vi "Build CE Deploy - Create Project.vi"(8 "error in":errorcluster, 10 "Project Files":path[](array[path]), 11 "Target Dir":path) -> (0 "error out":errorcluster, 2 "Project File Path":path, 3 "dup Target Dir":path)   [LabVIEW 2021]
doc: "::: CalcExpress Toolkit :::\nCopyright (c) 2000-2026 Konstantin Shifershteyn. All rights reserved."
panel:
  # "CalcExpress Toolkit\nCopyright (c) 2000-2026 Konstantin Shifershteyn"
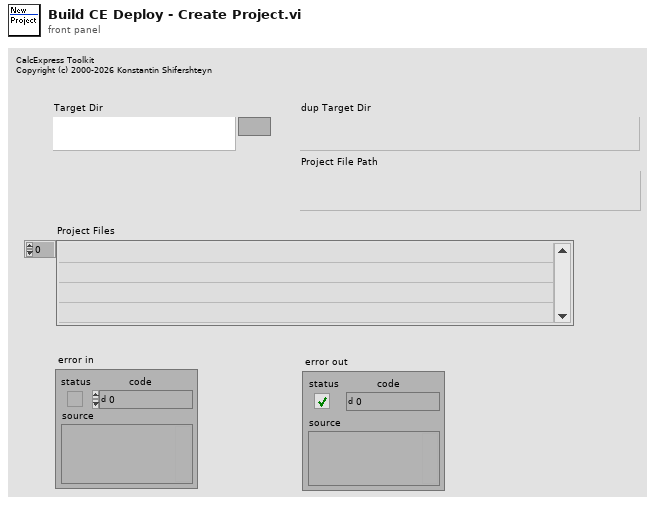
[diagram p1: front panel]
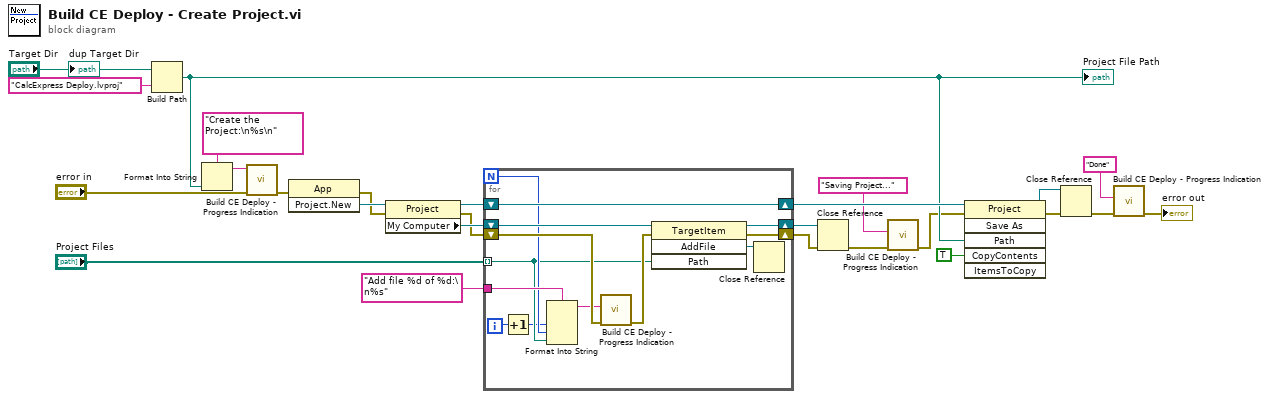
[diagram p0: block diagram]
diagram:
  n1 = Build Path(base path="Target Dir", name or relative path="CalcExpress Deploy.lvproj") -> (appended path=w7:path)
  "Project File Path" <- w7
  n2 = Format Into String(format string="Create the Project:\n%s\n", w7) -> (resulting string=w9:string)  [unwired: 2 in, 1 out]
  n3 = call "Build CE Deploy - Progress Indication.vi"("error in"="error in", "message 1"=w9) -> ("error out"=w11:errorcluster)  [unwired: 9 in]
  n4 = invoke class="App" method="Project.New"(error in=w11) -> (error out=w22:errorcluster, "Project:New"=w24:refnum<vi>)  [unwired: 2 in, 1 out]
  n5 = property class="Project"(reference=w24, error in=w22) -> (reference out=w26:refnum<vi>, error out=w20:errorcluster, "My Computer"=w23:refnum<vi>)
  n6 = for {
    N -> [w30]
    tunnel: "Project Files" -> [w29] mode=indexing
    shift-right: [w38] -> w21
    shift-left: w23 -> [w39]
    shift-right: [w36] -> w25
    shift-left: w20 -> [w34]
    shift-right: [w35] -> w14
    shift-left: w26 -> [w35]
    tunnel: "Add file %d of %d:\n%s" -> [w32]
    i -> [w31]
    n7 = Increment(x=w31) -> (x+1=w28:i32)
    n8 = Format Into String(format string=w32, w28, w30, w29) -> (resulting string=w27:string)  [unwired: 2 in, 1 out]
    n9 = call "Build CE Deploy - Progress Indication.vi"("error in"=w34, "message 2"=w27) -> ("error out"=w33:errorcluster)  [unwired: 9 in]
    n10 = invoke class="TargetItem" method="AddFile"(reference=w39, error in=w33, "Path"=w29) -> (reference out=w38:refnum<vi>, error out=w36:errorcluster, "AddFile"=w37:refnum<vi>)  [unwired: 1 in, 1 out]
    n11 = Close Reference(reference=w37) -> ()  [unwired: 1 in, 1 out]
  }
  n12 = Close Reference(reference=w21, error in (no error)=w25) -> (error out=w6:errorcluster)
  n13 = call "Build CE Deploy - Progress Indication.vi"("error in"=w6, "message 2"="Saving Project...") -> ("error out"=w5:errorcluster)  [unwired: 9 in]
  n14 = invoke class="Project" method="Save As"(reference=w14, error in=w5, "Path"=w7, "CopyContents"=TRUE ("Copy contents?")) -> (reference out=w17:refnum<vi>, error out=w18:errorcluster)  [unwired: 2 in, 4 out]
  n15 = Close Reference(reference=w17, error in (no error)=w18) -> (error out=w3:errorcluster)
  n16 = call "Build CE Deploy - Progress Indication.vi"("error in"=w3, "message 2"="Done") -> ("error out"=→"error out":errorcluster)  [unwired: 9 in]
  "dup Target Dir" <- "Target Dir"
